vi "UI Convert Map to Listbox.vi"(10 "Byte spaces":u32=1, 11 "CAN Return MAP in":T1 {"CAN frame"."payload" format="%x"; "CAN frame"."timestamp" format="%<%.7X\n%x>T"; "CAN frame"."type" items=["CAN Data"=0, "CAN Remote"=1, "CAN Bus Error"=2, "CAN 2.0 Data"=8, "CAN FD Data"=16, "CAN FD+BRS Data"=24, "J1939 Data"=192, "Delay"=224, "Log Trigger"=225, "Start Trigger"=226]; "CAN frame"."identifier" format="%x"}) -> (3 "CAN Data for Mutli Listbox":string[][](array[string]))   [LabVIEW 2021, in "XNET CAN RW.lvclass"]
doc: "Create text for listbox. Listbox is intended for headers of ID, Timestamp, Payload. Payload is displayed in hex format and the spacing between bytes is configurable."
uses:
  XNET CAN RW.lvclass
  typedef/CAN Return Map.ctl
  <vilib>/xnet/xnet.llb/XNET Frame CAN.ctl
  <vilib>/xnet/xnet.llb/XNET Frame Type CAN.ctl
panel:
  out "Plugin Status":string[][](table)
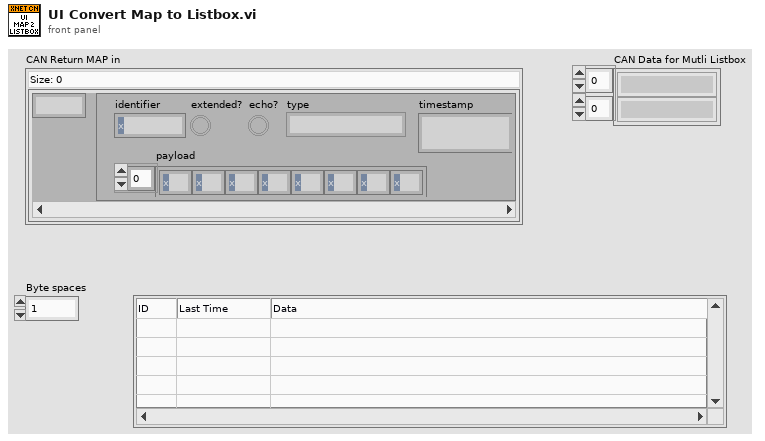
[diagram p1: front panel]
types:
  T1 = typedef "XNET CAN RW.lvclass/CAN Return Map.ctl" = map{u32, T2}
  T2 = typedef "XNET Frame CAN.ctl" = cluster{"timestamp":timestamp, "payload":u8[], "identifier":u32, "type":T3, "extended?":bool, "echo?":bool}
  T3 = typedef "XNET Frame Type CAN.ctl" = u8
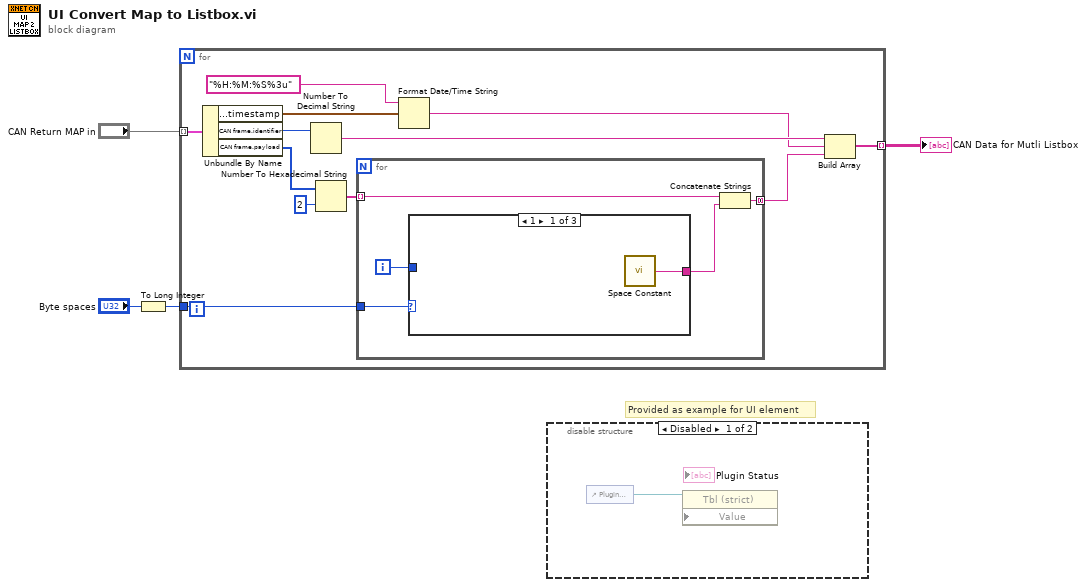
[diagram p0: block diagram]
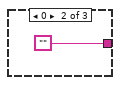
[diagram p3: hidden frame]
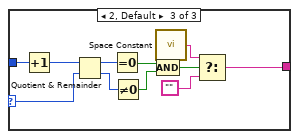
[diagram p4: hidden frame]
diagram:
  # "Provided as example for UI element"
  n1 = To Long Integer(number="Byte spaces") -> (32bit integer=w1:i32)
  n2 = for {
    tunnel: "CAN Return MAP in" -> [w16] mode=indexing
    tunnel: [w13] -> w4 mode=indexing
    tunnel: w1 -> [w5]
    n3 = Unbundle By Name(w16) -> ("CAN frame.timestamp"=w10:timestamp, "CAN frame.identifier"=w15:u32, "CAN frame.payload"=w8:u8[])
    n4 = Number To Decimal String(number=w15) -> (decimal integer string=w14:string)  [unwired: 1 in]
    n5 = Number To Hexadecimal String(1:i16 2 ("width (-)"), 2:w8) -> (0:w7:string[])
    n6 = for {
      tunnel: [w20] -> w12 mode=concatenating
      tunnel: w7 -> [w19] mode=indexing
      tunnel: w5 -> [w17]
      i -> [w21]
      n7 = case shown="1" w17 {
        selector: w17 -> [_ _ w24]
        tunnel: w21 -> [_ _ w34]
        tunnel: [w22 "" w33] -> w18
        frame 1 {
          n8 = call <vilib>:"Space Constant.vi"() -> ("String"=w22:string)
        }
        frame 0 {
        }
        frame 2, Default {
          n9 = Increment(x=w34) -> (x+1=w26:i32)
          n10 = Quotient & Remainder(x=w26, y=w24) -> (x-y*floor(x/y)=w32:i32, floor(x/y)=w31:i32)
          n11 = Equal To 0?(x=w32) -> (x = 0?=w30:bool)
          n12 = Not Equal To 0?(x=w31) -> (x != 0?=w29:bool)
          n13 = call <vilib>:"Space Constant.vi"() -> ("String"=w25:string)
          n14 = Compound Arithmetic op=AND(w30, w29) -> (w28:bool)
          n15 = Select(t=w25, s=w28, f="") -> (s? t:f=w33:string)
        }
      }
      n16 = Concatenate Strings(w19, w18) -> (w20:string)
    }
    n17 = Format Date/Time String(time format string (%c)="%H:%M:%S%3u", seconds (now)=w10) -> (date/time string=w9:string)  [unwired: 1 in]
    n18 = Build Array(w14, w9, w12) -> (w13:string[])
  }
  "CAN Data for Mutli Listbox" <- w4
  n19 = disable-structure shown="Disabled" {
    frame Disabled {
      n20 = control-ref of="Plugin Status"() -> (w35:refnum<vi>)
      n21 = property class="Tbl (strict)" props=["Value"](reference=w35) -> ()  [unwired: 2 in, 2 out]
    }
    frame Enabled {
    }
  }
